vi "Wrapper For Assert True.vi"(8 "error in (no error)":errorcluster) -> (0 "error out":errorcluster)   [LabVIEW 2020]
uses:
  classes/Assert/Assert.lvclass
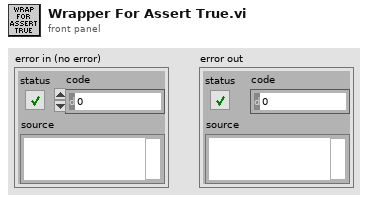
[diagram p1: front panel]
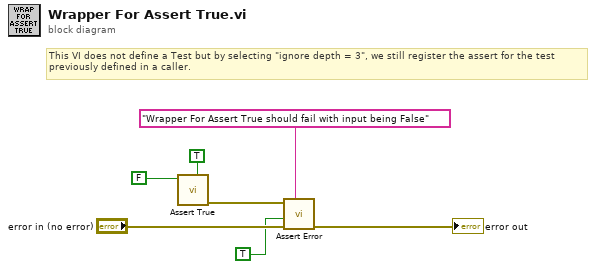
[diagram p0: block diagram]
diagram:
  # "This VI does not define a Test but by selecting \"ignore depth = 3\", we still register the assert for the test\npreviously defined in a caller."
  n1 = call "Assert True.vi"("Assert Only? (F)"=TRUE, "True?"=FALSE) -> ("error out"=w4:errorcluster)  [unwired: 8 in, 1 out]
  n2 = call "Assert Error.vi"("Label"="Wrapper For Assert True should fail with input being False", "error in (no error)"="error in (no error)", "Register with caller test (F)"=TRUE, "Error?"=w4) -> ("error out"=→"error out":errorcluster)  [unwired: 6 in, 1 out]
